vi "Get T1Status.vi"(0 "uXMax":u32, 1 "strFileName":string, 5 "uXLastNoZeroValue":u32, 7 "uYMax":u64, 9 "uCount":u32, 11 "error in (no error)":errorcluster caption="错误输入（无错误）") -> (3 "strFileName out":string, 4 "uXMax out":u32, 6 "uXLastNoZeroValue out":u32, 8 "uYMax 2":u64, 10 "uCount out":u32, 14 "function return":i32, 15 "error out":errorcluster caption="错误输出")   [LabVIEW 2017, in "smncsftmt.lvlib"]
doc: "__declspec(dllexport) int GetT1Status(unsigned int* uXMax, unsigned int* uXLastNoZeroValue, unsigned long long* uYMax, unsigned int* uCount, char* strFileName);"
uses:
  smncsftmt.lvlib
  smncsftmt.dll
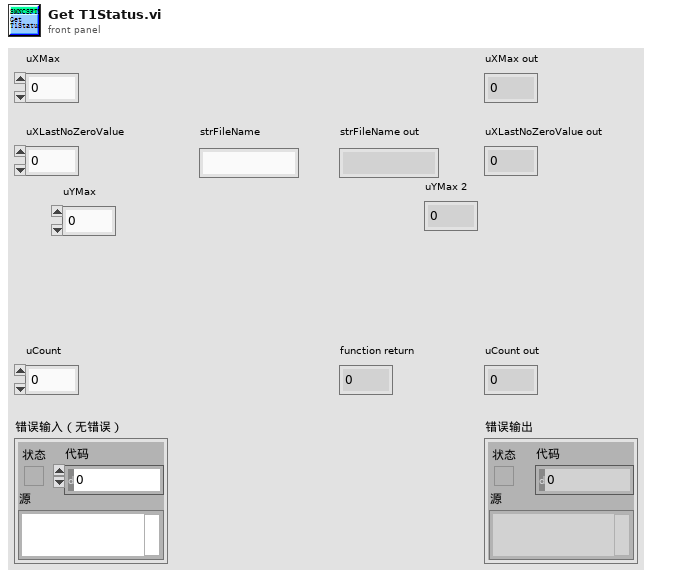
[diagram p1: front panel]
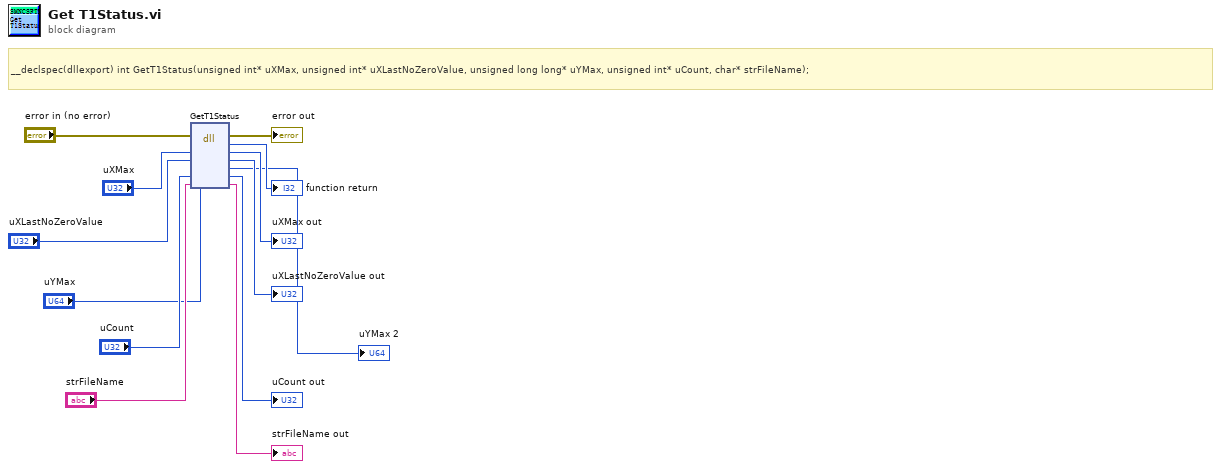
[diagram p0: block diagram]
diagram:
  # "__declspec(dllexport) int GetT1Status(unsigned int* uXMax, unsigned int* uXLastNoZeroValue, unsigned long long* uYMax, unsigned int* uCount, char* strFileName);"
  n1 = dll-call lib="PTH2oabs CUsersaDesktop\nLABVIEW范例National InstrumentsLabVIEW 2017user.lib\tsmncsftmtsmncsftmt.*" fn="GetT1Status"(error in="error in (no error)", "uXMax"="uXMax", "uXLastNoZeroValue"="uXLastNoZeroValue", "uYMax"="uYMax", "uCount"="uCount", "strFileName"="strFileName") -> (error out=→"error out":errorcluster, "返回类型"=→"function return":i32, "uXMax"=→"uXMax out":u32, "uXLastNoZeroValue"=→"uXLastNoZeroValue out":u32, "uYMax"=→"uYMax 2":u64, "uCount"=→"uCount out":u32, "strFileName"=→"strFileName out":string)  [unwired: 2 in, 1 out]
